vi "Test Load Waveform from TDMS.vi"(8 "error in (no error)":errorcluster) -> (0 "error out":errorcluster)   [LabVIEW 2016]
uses:
  <vilib>/addons/_JKI Toolkits/Caraya/classes/Assert/Assert True.vi
  <vilib>/addons/_JKI Toolkits/Caraya/classes/Assert/Assert Less Or Equal_Variant.vi
  <vilib>/addons/_JKI Toolkits/Caraya/classes/Assert/Assert Almost Equal_Float.vi
  <vilib>/addons/_JKI Toolkits/Caraya/classes/Assert/Assert False.vi
  <vilib>/addons/_JKI Toolkits/Caraya/classes/Assert/Assert Greater_Variant.vi
  <vilib>/addons/_JKI Toolkits/Caraya/classes/Assert/Assert Greater Or Equal_Variant.vi
  <instrlib>/niRFSGPlayback/niRFSGPlayback Download User Waveform (CSG).vi
  <vilib>/addons/_JKI Toolkits/Caraya/classes/Assert/Assert Equal Value_Variant.vi
  <vilib>/Utility/config.llb/Read Key (Boolean).vi
  Source/SG/SG.lvlib
  <vilib>/addons/_JKI Toolkits/Caraya/classes/Test/Test.lvclass
  <vilib>/addons/_JKI Toolkits/Caraya/classes/Assert/Assert.lvclass
  <vilib>/Utility/config.llb/NI_LVConfig.lvlib
  Source/Common/Common.lvlib
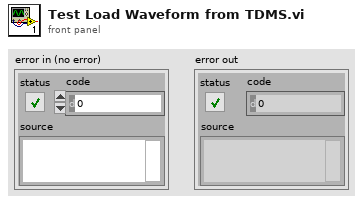
[diagram p1: front panel]
types:
  T1 = enum16{"Waveform.dx greater than 0", "Waveform.y not empty", "Waveform.dx equal to 1/fs", "Sample rate greater than 0", "Signal bandwidth geq to 0", "Burst length greater than 0", "Papr geq to 0", "Start locations not empty", "Stop locations not empty", "Runtime scaling leq to 0", "Entire waveform read", "Papr agrees with playback library calculation", "Idle duration present calculated correctly", "Waveform read from library matches loaded type"}
  T2 = typedef "Common.lvlib/Waveform.ctl" = cluster{"Name":string, "Data":refnum<data-value>, "Signal Bandwidth (Hz)":dbl, "PAPR (dB)":dbl, "Burst Length (s)":dbl, "Sample Rate":dbl, "Burst Start Locations":i32[], "Burst Stop Locations":i32[], "Idle Duration Present?":bool, "Runtime Scaling":dbl, "Script":string}
  T3 = typedef "NI_LVConfig.lvlib/Config Data RefNum.ctl" = refnum<k1>
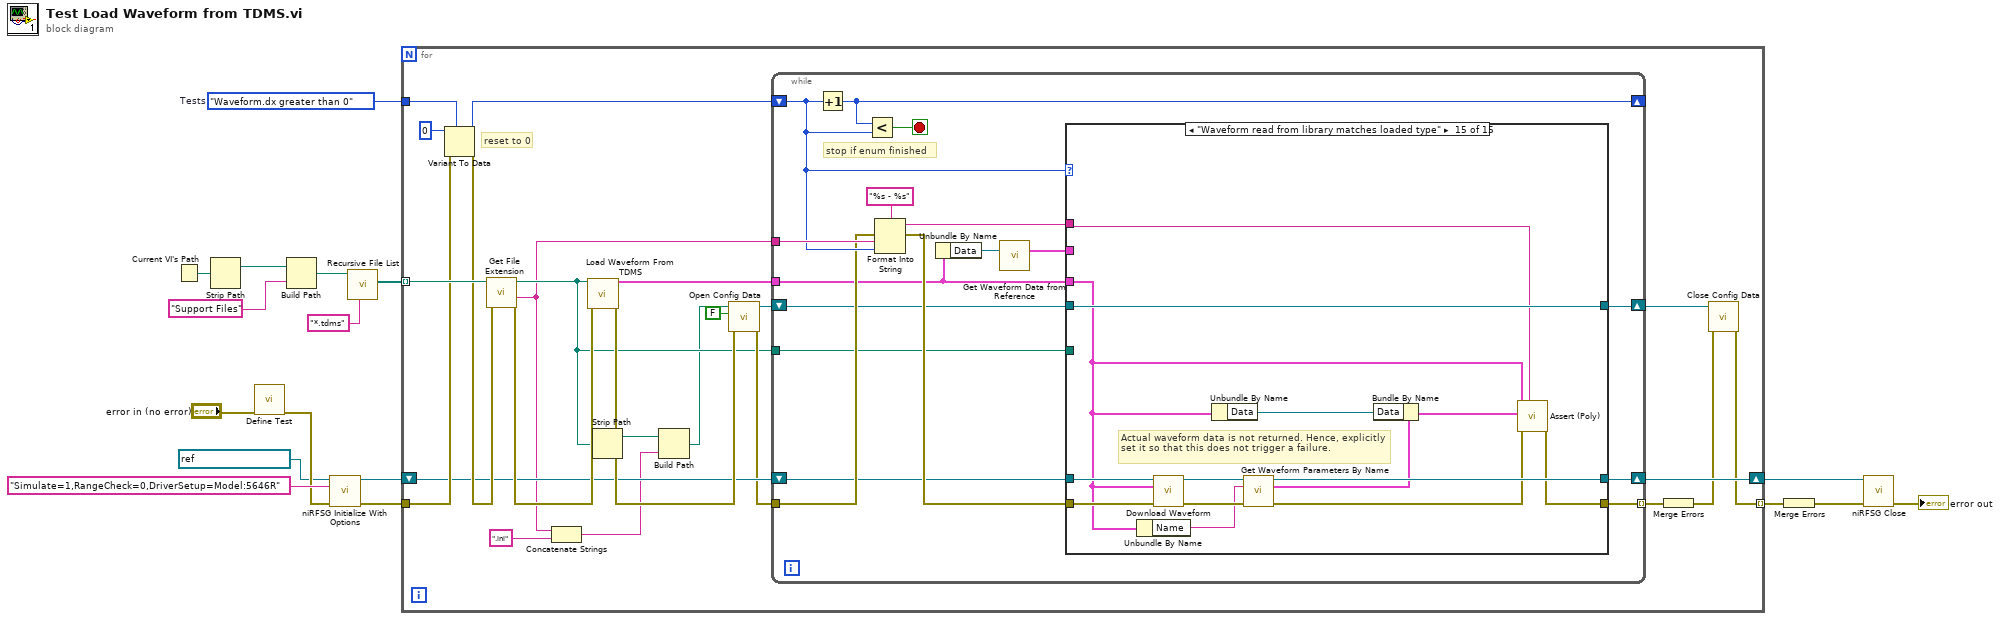
[diagram p0: block diagram]
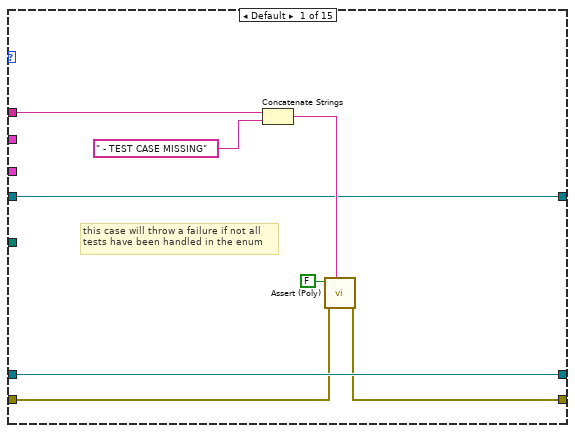
[diagram p2: hidden frame]
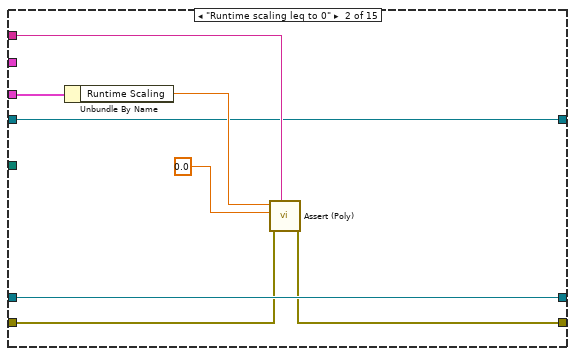
[diagram p3: hidden frame]
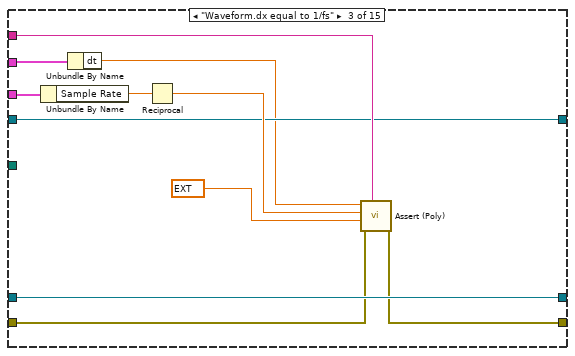
[diagram p4: hidden frame]
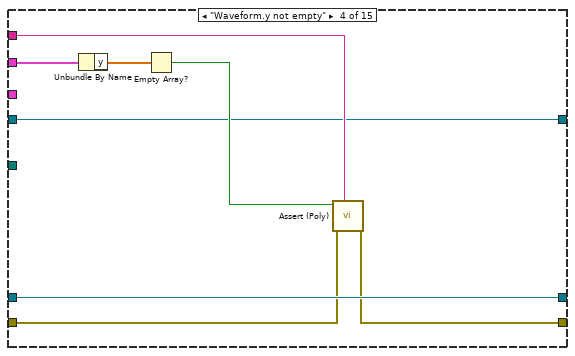
[diagram p5: hidden frame]
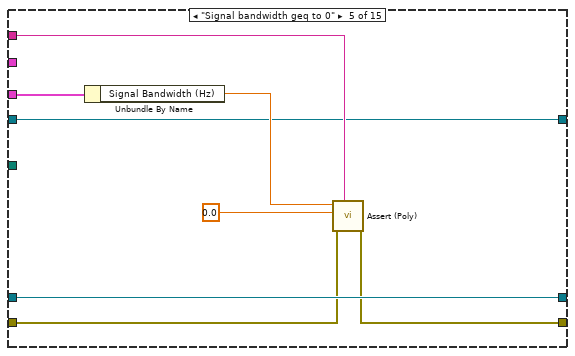
[diagram p6: hidden frame]
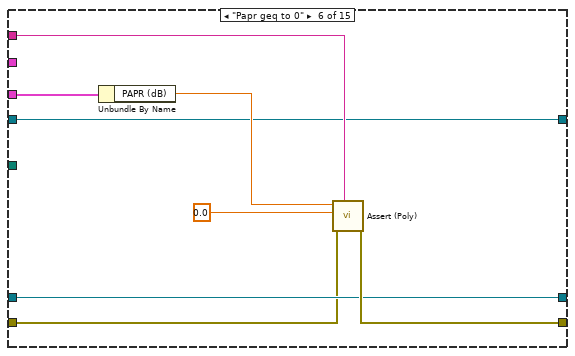
[diagram p7: hidden frame]
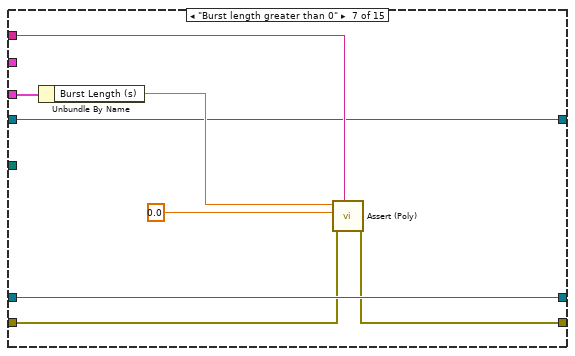
[diagram p8: hidden frame]
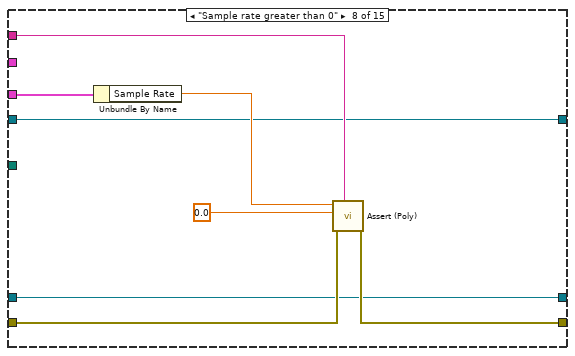
[diagram p9: hidden frame]
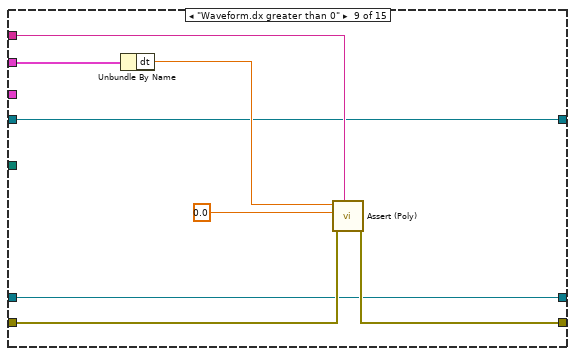
[diagram p10: hidden frame]
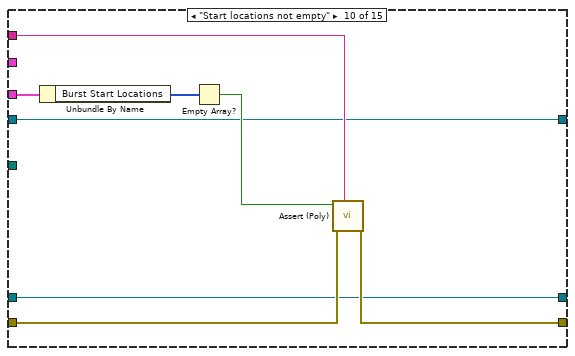
[diagram p11: hidden frame]
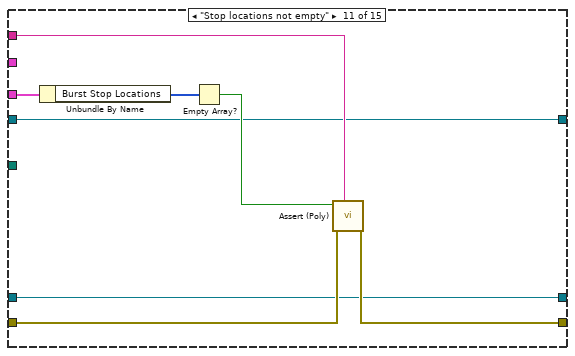
[diagram p12: hidden frame]
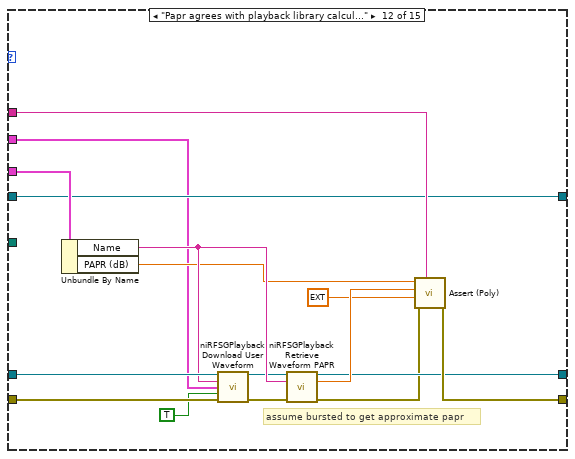
[diagram p13: hidden frame]
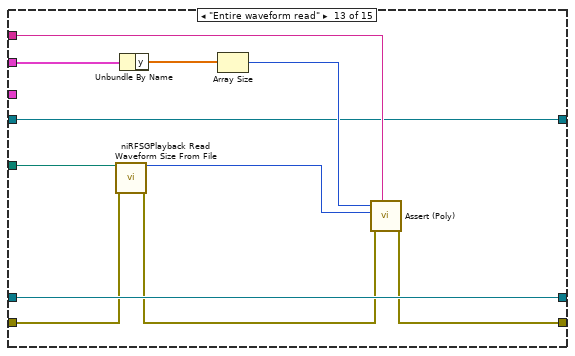
[diagram p14: hidden frame]
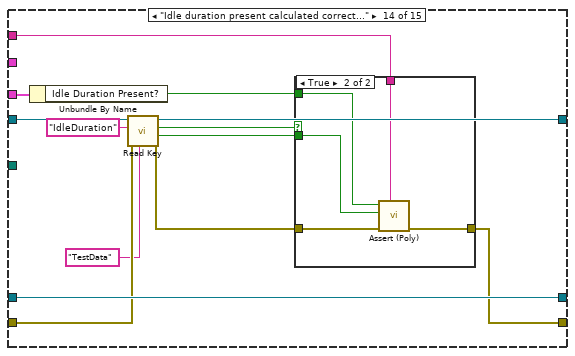
[diagram p15: hidden frame]
diagram:
  w9 = T1."Waveform.dx greater than 0"  # Tests
  n1 = Current VI's Path() -> (path=w17:path)
  n2 = Strip Path(path=w17) -> (stripped path=w16:path)  [unwired: 1 out]
  n3 = call <vilib>:"Define Test.vi"("error in (no error)"="error in (no error)") -> ("error out"=w6:errorcluster)  [unwired: 10 in]
  n4 = Build Path(base path=w16, name or relative path="Support Files") -> (appended path=w12:path)
  n5 = call <instrlib>:"niRFSG Initialize With Options.vi"("resource name"=refnum<k15> "SimulatedDevice", "option string"="Simulate=1,RangeCheck=0,DriverSetup=Model:5646R", "error in"=w6) -> ("instrument handle"=w7:refnum<k15>, "error out"=w5:errorcluster)  [unwired: 11 in]
  n6 = call <vilib>:"Recursive File List.vi"("pattern"="*.tdms", "Folder Path"=w12) -> ("All Files in Dir"=w11:path[])  [unwired: 5 in, 4 out]
  n7 = for {
    tunnel: w11 -> [w38] mode=indexing
    tunnel: w5 -> [w33]
    tunnel: [w18] -> w10 mode=indexing
    tunnel: w9 -> [w36]
    shift-right: [w30] -> w2
    shift-left: w7 -> [w31]
    # "reset to 0"
    n8 = Variant To Data(error in=w33, type=w36, Variant=i16 0) -> (data=w34:T1, error out=w32:errorcluster)
    n9 = call <vilib>:"Get File Extension.vi"("error in (no error)"=w32, "file"=w38) -> ("error out"=w37:errorcluster, "filename without extension"=w23:string, "dup file"=w26:path)  [unwired: 5 in, 2 out]
    n10 = Concatenate Strings(w23, ".ini" ("string")) -> (w24:string)
    n11 = call "Load Waveform From TDMS.vi"("TDMS File Path"=w26, "error in (no error)"=w37) -> ("Waveform"=w40:T2, "error out"=w41:errorcluster)  [unwired: 12 in]
    n12 = Strip Path(path=w26) -> (stripped path=w25:path)  [unwired: 1 out]
    n13 = Build Path(base path=w25, name or relative path=w24) -> (appended path=w21:path)
    n14 = call <vilib>:"Open Config Data.vi"("error in (no error)"=w41, "create file if necessary (T)"=FALSE, "configuration file path"=w21) -> ("error out"=w27:errorcluster, "refnum"=w29:T3)  [unwired: 6 in, 1 out]
    n15 = while {
      tunnel: w40 -> [w44]
      tunnel: [w46] -> w39 mode=indexing
      tunnel: w23 -> [w57]
      shift-right: [w55] -> _
      shift-left: w34 -> [w54]
      tunnel: w27 -> [w52]
      shift-right: [w50] -> w30
      shift-left: w31 -> [w51]
      tunnel: w26 -> [w49]
      shift-right: [w45] -> w20
      shift-left: w29 -> [w47]
      stop <- w48 stop-if-true
      # "stop if enum finished"
      n16 = Increment(x=w54) -> (x+1=w55:T1)
      n17 = Less?(x=w55, y=w54) -> (x < y?=w48:bool)
      n18 = Format Into String(format string="%s - %s", error in=w52, w57, w54) -> (resulting string=w56:string, error out=w53:errorcluster)  [unwired: 1 in]
      n19 = Unbundle By Name(w44) -> ("Data"=w43:refnum<data-value>)
      n20 = call "Get Waveform Data from Reference.vi"("Waveform Data Reference"=w43) -> ("Waveform Data"=w42:cluster{"t0":dbl, "dt":dbl, "y":csg[]})  [unwired: 13 in, 1 out]
      n21 = case shown="\"Waveform read from library matches loaded type\"" w54 {
        tunnel: [w59 w67 w77 w88 w94 w109 w110 w125 w133 w141 w149 w162 w172 w182 w197] -> w46
        tunnel: w44 -> [_ w74 w85 _ w101 w108 w117 w124 _ w140 w148 w164 _ w178 w200]
        tunnel: w56 -> [w64 w71 w81 w92 w98 w105 w114 w121 w130 w137 w145 w158 w171 w181 w199]
        tunnel: w53 -> [w60 w68 w78 w89 w95 w102 w111 w120 w129 w136 w144 w157 w174 w186 w207]
        tunnel: w51 -> [w66 w70 w80 w91 w97 w104 w113 w119 w128 w135 w143 w165 w176 w189 w208]
        tunnel: [w66 w70 w80 w91 w97 w104 w113 w119 w128 w135 w143 w159 w176 w189 w204] -> w50
        tunnel: w49 -> [_ _ _ _ _ _ _ _ _ _ _ _ w175 _ _]
        tunnel: w47 -> [w61 w69 w79 w90 w96 w103 w112 w118 w127 w134 w142 w154 w167 w188 w209]
        tunnel: [w61 w69 w79 w90 w96 w103 w112 w118 w127 w134 w142 w154 w167 w187 w209] -> w45
        tunnel: w42 -> [_ _ w76 w87 _ _ _ _ w126 _ _ w150 w166 _ _]
        frame Default {
          # "this case will throw a failure if not all\ntests have been handled in the enum"
          n22 = Concatenate Strings(w64, " - TEST CASE MISSING" ("Label")) -> (w62:string)
          n23 = call-poly <vilib>:"Assert (Poly).vi"("Label"=w62, "error in (no error)"=w60, "True?"=FALSE) -> ("error out"=w59:errorcluster)  [unwired: 8 in]
        }
        frame "Runtime scaling leq to 0" {
          n24 = Unbundle By Name(w74) -> ("Runtime Scaling"=w73:dbl)
          n25 = call-poly <vilib>:"Assert (Poly).vi"("Label"=w71, "error in (no error)"=w68, "Y"=0.0 ("Runtime Scaling"), "X"=w73) -> ("error out"=w67:errorcluster)  [unwired: 7 in]
        }
        frame "Waveform.dx equal to 1/fs" {
          n26 = Unbundle By Name(w85) -> ("Sample Rate"=w84:dbl)
          n27 = Unbundle By Name(w76) -> ("dt"=w75:dbl)
          n28 = Reciprocal(x=w84) -> (1/x=w83:dbl)
          n29 = call-poly <vilib>:"Assert (Poly).vi"("Label"=w81, "error in (no error)"=w78, "Tolerance"=ext 0.00099999999999999999996, "Y"=w83, "X"=w75) -> ("error out"=w77:errorcluster)  [unwired: 6 in]
        }
        frame "Waveform.y not empty" {
          n30 = Unbundle By Name(w87) -> ("y"=w86:csg[])
          n31 = Empty Array?(array=w86) -> (empty?=w93:bool)
          n32 = call-poly <vilib>:"Assert (Poly).vi"("Label"=w92, "error in (no error)"=w89, "False?"=w93) -> ("error out"=w88:errorcluster)  [unwired: 8 in]
        }
        frame "Signal bandwidth geq to 0" {
          n33 = Unbundle By Name(w101) -> ("Signal Bandwidth (Hz)"=w100:dbl)
          n34 = call-poly <vilib>:"Assert (Poly).vi"("Label"=w98, "error in (no error)"=w95, "Y"=0.0 ("Signal Bandwidth (Hz)"), "X"=w100) -> ("error out"=w94:errorcluster)  [unwired: 7 in]
        }
        frame "Papr geq to 0" {
          n35 = Unbundle By Name(w108) -> ("PAPR (dB)"=w107:dbl)
          n36 = call-poly <vilib>:"Assert (Poly).vi"("Label"=w105, "error in (no error)"=w102, "Y"=0.0 ("Signal Bandwidth (Hz)"), "X"=w107) -> ("error out"=w109:errorcluster)  [unwired: 7 in]
        }
        frame "Burst length greater than 0" {
          n37 = Unbundle By Name(w117) -> ("Burst Length (s)"=w116:dbl)
          n38 = call-poly <vilib>:"Assert (Poly).vi"("Label"=w114, "error in (no error)"=w111, "Y"=0.0 ("Signal Bandwidth (Hz)"), "X"=w116) -> ("error out"=w110:errorcluster)  [unwired: 7 in]
        }
        frame "Sample rate greater than 0" {
          n39 = Unbundle By Name(w124) -> ("Sample Rate"=w123:dbl)
          n40 = call-poly <vilib>:"Assert (Poly).vi"("Label"=w121, "error in (no error)"=w120, "Y"=0.0 ("Signal Bandwidth (Hz)"), "X"=w123) -> ("error out"=w125:errorcluster)  [unwired: 7 in]
        }
        frame "Waveform.dx greater than 0" {
          n41 = Unbundle By Name(w126) -> ("dt"=w132:dbl)
          n42 = call-poly <vilib>:"Assert (Poly).vi"("Label"=w130, "error in (no error)"=w129, "Y"=0.0 ("Signal Bandwidth (Hz)"), "X"=w132) -> ("error out"=w133:errorcluster)  [unwired: 7 in]
        }
        frame "Start locations not empty" {
          n43 = Unbundle By Name(w140) -> ("Burst Start Locations"=w139:i32[])
          n44 = Empty Array?(array=w139) -> (empty?=w138:bool)
          n45 = call-poly <vilib>:"Assert (Poly).vi"("Label"=w137, "error in (no error)"=w136, "False?"=w138) -> ("error out"=w141:errorcluster)  [unwired: 8 in]
        }
        frame "Stop locations not empty" {
          n46 = Unbundle By Name(w148) -> ("Burst Stop Locations"=w147:i32[])
          n47 = Empty Array?(array=w147) -> (empty?=w146:bool)
          n48 = call-poly <vilib>:"Assert (Poly).vi"("Label"=w145, "error in (no error)"=w144, "False?"=w146) -> ("error out"=w149:errorcluster)  [unwired: 8 in]
        }
        frame "Papr agrees with playback library calculation" {
          # "assume bursted to get approximate papr"
          n49 = Unbundle By Name(w164) -> ("Name"=w163:string, "PAPR (dB)"=w161:dbl)
          n50 = call-poly <instrlib>:"niRFSGPlayback Download User Waveform.vi"("instrument handle in"=w165, "waveform name"=w163, "waveform in"=w150, "burst present"=TRUE, "error in"=w157) -> ("instrument handle out"=w153:refnum<k15>, "error out"=w152:errorcluster)  [unwired: 9 in]
          n51 = call <instrlib>:"niRFSGPlayback Retrieve Waveform PAPR.vi"("instrument handle in"=w153, "waveform name"=w163, "error in"=w152) -> ("instrument handle out"=w159:refnum<k15>, "PAPR"=w160:dbl, "error out"=w156:errorcluster)  [unwired: 10 in]
          n52 = call-poly <vilib>:"Assert (Poly).vi"("Label"=w158, "error in (no error)"=w156, "Tolerance"=ext 0.1, "Y"=w160, "X"=w161) -> ("error out"=w162:errorcluster)  [unwired: 6 in]
        }
        frame "Entire waveform read" {
          n53 = call <instrlib>:"niRFSGPlayback Read Waveform Size From File.vi"("file path"=w175, "error in"=w174) -> ("waveform size"=w168:i32, "error out"=w173:errorcluster)  [unwired: 12 in]
          n54 = Unbundle By Name(w166) -> ("y"=w170:csg[])
          n55 = Array Size(array=w170) -> (size(s)=w169:i32)
          n56 = call-poly <vilib>:"Assert (Poly).vi"("Label"=w171, "error in (no error)"=w173, "Y"=w168, "X"=w169) -> ("error out"=w172:errorcluster)  [unwired: 7 in]
        }
        frame "Idle duration present calculated correctly" {
          n57 = Unbundle By Name(w178) -> ("Idle Duration Present?"=w177:bool)
          n58 = call-poly <vilib>:"Read Key.vi"("section"="TestData", "error in (no error)"=w186, "key"="IdleDuration", "refnum"=w188) -> ("error out"=w185:errorcluster, "value"=w179:bool, "found?"=w180:bool, "refnum out"=w187:T3)  [unwired: 4 in]
          n59 = case shown="True" w180 {
            tunnel: w185 -> [w190 w195]
            tunnel: [w190 w194] -> w182
            tunnel: w181 -> [_ w193]
            tunnel: w179 -> [_ w192]
            tunnel: w177 -> [_ w191]
            frame False {
              # "Don't run test if key not found"
            }
            frame True {
              n60 = call-poly <vilib>:"Assert (Poly).vi"("Label"=w193, "error in (no error)"=w195, "Y"=w192, "X"=w191) -> ("error out"=w194:errorcluster)  [unwired: 7 in]
            }
          }
        }
        frame "Waveform read from library matches loaded type" {
          # "Actual waveform data is not returned. Hence, explicitly set it so that this does not trigger a failure."
          n61 = Unbundle By Name(w200) -> ("Name"=w203:string)
          n62 = call "Download Waveform.vi"("RFSG handle"=w208, "Waveform In"=w200, "error in (no error)"=w207) -> ("RFSG handle out"=w206:refnum<k15>, "error out"=w205:errorcluster)  [unwired: 11 in]
          n63 = Unbundle By Name(w200) -> ("Data"=w196:refnum<data-value>)
          n64 = call "Get Waveform Parameters By Name.vi"("RFSG handle"=w206, "Waveform Name"=w203, "error in (no error)"=w205) -> ("RFSG handle out"=w204:refnum<k15>, "Waveform"=w202:T2, "error out"=w198:errorcluster)  [unwired: 10 in]
          n65 = Bundle By Name(cluster=w202, "Data"=w196) -> (w201:T2)
          n66 = call-poly <vilib>:"Assert (Poly).vi"("Label"=w199, "error in (no error)"=w198, "Y"=w201, "X"=w200) -> ("error out"=w197:errorcluster)  [unwired: 7 in]
        }
      }
    }
    n67 = Merge Errors(w39) -> (w19:errorcluster)
    n68 = call <vilib>:"Close Config Data.vi"("error in (no error)"=w19, "refnum"=w20) -> ("error out"=w18:errorcluster)  [unwired: 8 in, 1 out]
  }
  n69 = Merge Errors(w10) -> (w3:errorcluster)
  n70 = call <instrlib>:"niRFSG Close.vi"("instrument handle"=w2, "error in"=w3) -> ("error out"=→"error out":errorcluster)  [unwired: 13 in]
